vi "Write Numeric Outputs.vi"(8 "error in (no error)":errorcluster, 11 "Modbus in":refnum<class "Modbus.lvclass">) -> (0 "error out":errorcluster, 3 "Modbus out":refnum<class "Modbus.lvclass">)   [LabVIEW 2026, in "Modbus.lvlib" / "Modbus.lvclass"]
uses:
  Modbus.lvclass
  Modbus.lvclass/Modbus.ctl
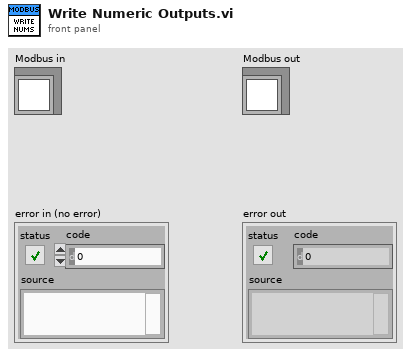
[diagram p1: front panel]
types:
  T1 = typedef "Modbus.lvlib/Modbus.lvclass/Numeric Data.ctl" = cluster{"Channel UID":string, "Valid?":bool, "Table":T2, "Address":i32, "Quantity":u16, "Size":T3, "Data Type":T4, "Location":T5}
  T2 = typedef "Modbus.lvlib/Modbus.lvclass/Modbus Table.ctl" = enum16{"Discrete Inputs", "Coils", "Input Registers", "Holding Registers"}
  T3 = typedef "Modbus.lvlib/Modbus.lvclass/Numeric Size.ctl" = enum16{"8-bit (Half register)", "16-bit (One register)", "32-bit (Two registers)", "64-bit (Four registers)"}
  T4 = typedef "Modbus.lvlib/Modbus.lvclass/Numeric Data Type.ctl" = enum16{"Unsigned Integer", "Signed Integer", "Floating Point"}
  T5 = typedef "Modbus.lvlib/Modbus.lvclass/Numeric Location.ctl" = enum16{"Low Byte", "High Byte"}
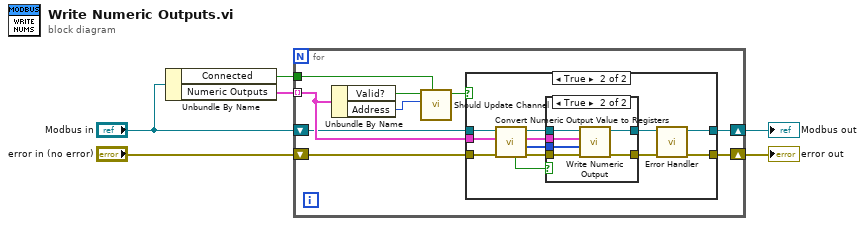
[diagram p0: block diagram]
diagram:
  n1 = Unbundle By Name("Modbus in") -> ("Connected"=w1:bool, "Numeric Outputs"=w2:T1[])
  n2 = for {
    tunnel: w2 -> [w15] mode=indexing
    shift-right: [w10] -> w6
    shift-left: "error in (no error)" -> [w13]
    tunnel: w1 -> [w11]
    shift-right: [w8] -> w3
    shift-left: "Modbus in" -> [w9]
    n3 = Unbundle By Name(w15) -> ("Valid?"=w12:bool, "Address"=w7:i32)
    n4 = call "Should Update Channel.vi"("Connected?"=w11, "Address"=w7, "Valid?"=w12) -> ("Update?"=w14:bool)  [unwired: 8 in]
    n5 = case shown="True" w14 {
      tunnel: [w17 w25] -> w10
      tunnel: w15 -> [_ w28]
      tunnel: w13 -> [w17 w27]
      tunnel: w9 -> [w16 w23]
      tunnel: [w16 w24] -> w8
      frame False {
      }
      frame True {
        n6 = call "Convert Numeric Output Value to Registers.vi"("error in (no error)"=w27, "Numeric Output in"=w28, "Plugin in"=w23) -> ("error out"=w29:errorcluster, "Register Values"=w19:u16[], "Numeric Output out"=w18:T1, "Plugin out"=w22:refnum<class "Modbus.lvclass">, "Data Valid"=w20:bool)  [unwired: 4 in]
        n7 = case shown="True" w20 {
          tunnel: [w31 w37] -> w26
          tunnel: w29 -> [w31 w36]
          tunnel: w19 -> [_ w35]
          tunnel: w22 -> [w30 w34]
          tunnel: [w30 w33] -> w21
          tunnel: w18 -> [_ w32]
          frame False {
          }
          frame True {
            n8 = call "Write Numeric Output.vi"("error in (no error)"=w36, "Register Values"=w35, "Numeric Output"=w32, "Modbus in"=w34) -> ("error out"=w37:errorcluster, "Modbus out"=w33:refnum<class "Modbus.lvclass">)  [unwired: 6 in]
          }
        }
        n9 = call "Error Handler.vi"("error in (no error)"=w26, "Modbus in"=w21) -> ("error out"=w25:errorcluster, "Modbus out"=w24:refnum<class "Modbus.lvclass">)  [unwired: 8 in]
      }
    }
  }
  "Modbus out" <- w3
  "error out" <- w6
